vi "command_current_producerconsumer__401e23a0a1.vi"(8 "error in (no error)":errorcluster, 9 "relative seconds":dbl, 10 "PID output":dbl, 11 "IVI Refnum in":refnum<k15>) -> (0 "error out":errorcluster, 2 "time stress":dbl, 3 "IVI Refnum out":refnum<k15>, 4 "current":dbl format="%_6g", 5 "voltage":dbl format="%_6g")   [LabVIEW 2023]
uses:
  <instrlib>/niDCPower/nidcpower.llb/niDCPower Measurement Type.ctl
panel:
  out "Measurement:Measure Record Delta Time":dbl
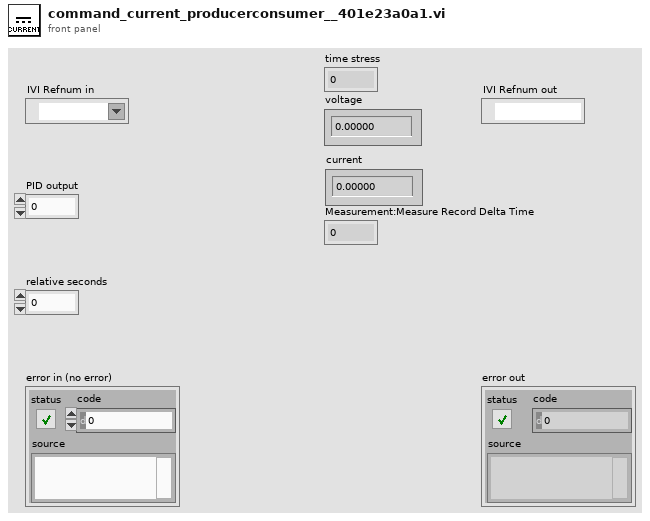
[diagram p1: front panel]
types:
  T1 = typedef "niDCPower Measurement Type.ctl" = i32
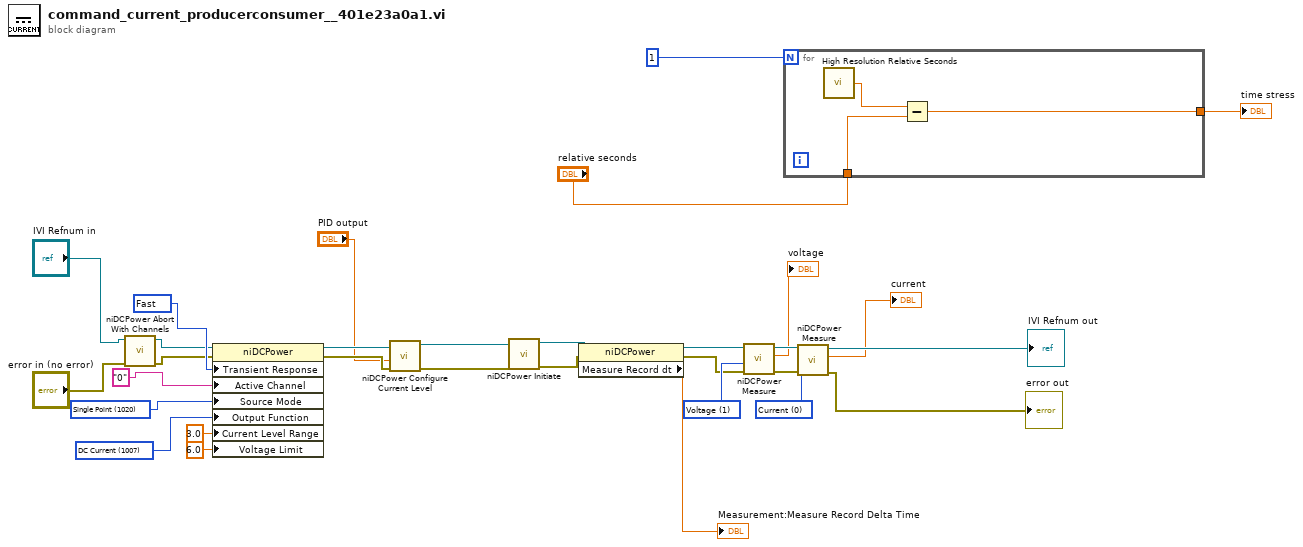
[diagram p0: block diagram]
diagram:
  w4 = T1 0 items=["Current", "Voltage"] ("measurement type")
  w6 = T1 1 items=["Current", "Voltage"] ("measurement type")
  w29 = 1007 items=["DC Voltage"=1006, "DC Current"=1007, "Pulse Voltage"=1049, "Pulse Current"=1050] ("Source:Output Function")
  w28 = 1020 items=["Single Point"=1020, "Sequence"=1021] ("Source:Source Mode")
  w16 = 1039 items=["Slow"=1041, "Normal"=1038, "Fast"=1039, "Custom"=1042] ("Source:Transient Response")
  n1 = call <instrlib>:"niDCPower Abort With Channels.vi"("error in (no error)"="error in (no error)", "instrument handle"="IVI Refnum in") -> ("error out"=w13:errorcluster, "instrument handle out"=w14:refnum<k15>)  [unwired: 8 in]
  n2 = property class="niDCPower"(reference=w14, error in=w13, "Transient Response"=w16, "Active Channel"="0", "Source Mode"=w28, "Output Function"=w29, "Current Level Range"=3.0 ("Source:DC Current:Current Level Range"), "Voltage Limit"=6.0 ("Source:DC Current:Voltage Limit")) -> (reference out=w20:refnum<k15>, error out=w21:errorcluster)
  n3 = call <instrlib>:"niDCPower Configure Current Level.vi"("error in (no error)"=w21, "current level"="PID output", "instrument handle"=w20) -> ("error out"=w27:errorcluster, "instrument handle out"=w26:refnum<k15>)  [unwired: 7 in]
  n4 = call <instrlib>:"niDCPower Initiate.vi"("error in (no error)"=w27, "instrument handle"=w26) -> ("error out"=w23:errorcluster, "instrument handle out"=w22:refnum<k15>)  [unwired: 2 in, 6 out]
  n5 = property class="niDCPower"(reference=w22, error in=w23) -> (reference out=w11:refnum<k15>, error out=w5:errorcluster, "Measure Record dt"=→"Measurement:Measure Record Delta Time":dbl)
  n6 = call <instrlib>:"niDCPower Measure.vi"("error in (no error)"=w5, "measurement type"=w6, "instrument handle"=w11) -> ("error out"=w7:errorcluster, "measurement"=→"voltage":dbl, "instrument handle out"=w10:refnum<k15>)  [unwired: 6 in]
  n7 = for {
    N: 1 -> [_]
    tunnel: "relative seconds" -> [w34]
    tunnel: [w32] -> w12
    n8 = call <vilib>:"High Resolution Relative Seconds.vi"() -> ("relative seconds"=w33:dbl)
    n9 = Subtract(x=w33, y=w34) -> (x-y=w32:dbl)
  }
  "time stress" <- w12
  n10 = call <instrlib>:"niDCPower Measure.vi"("error in (no error)"=w7, "measurement type"=w4, "instrument handle"=w10) -> ("error out"=→"error out":errorcluster, "measurement"=→"current":dbl, "instrument handle out"=→"IVI Refnum out":refnum<k15>)  [unwired: 6 in]
